vi "LabVIEW.Service.Log Rotating.vi"(6 "description":string, 7 "Command":T1(ring), 8 "error in (no error)":errorcluster caption="Fehler (Eingang, kein Fehler)", 9 "command":string, 10 "status":string, 11 "Pfad":path) -> (0 "error out":errorcluster caption="Fehler (Ausgang)")   [LabVIEW 2026]
uses:
  <vilib>/Utility/config.llb/Write Key (String).vi
  <vilib>/Utility/config.llb/NI_LVConfig.lvlib
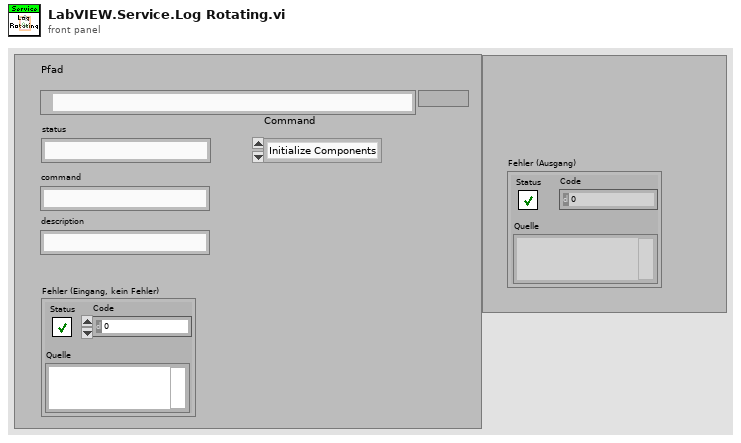
[diagram p1: front panel]
types:
  T1 = enum16{"Initialize Components", "Loging", "Delete Loging"}
  T2 = typedef "NI_LVConfig.lvlib/Config Data RefNum.ctl" = refnum<k1>
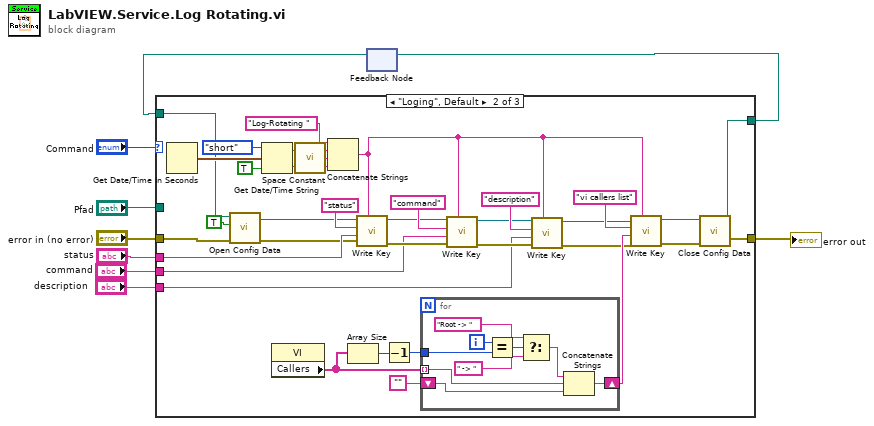
[diagram p0: block diagram]
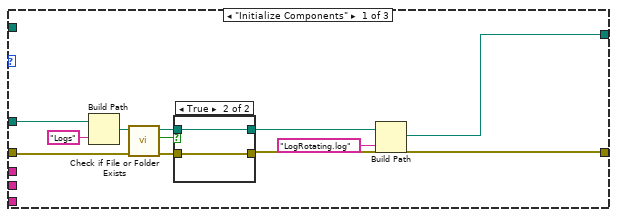
[diagram p2: hidden frame]
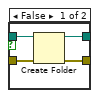
[diagram p3: hidden frame]
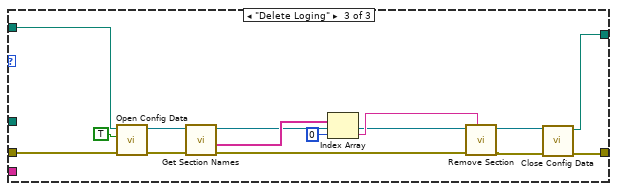
[diagram p4: hidden frame]
diagram:
  n1 = feedback #1() -> (w7:path)  [unwired: 1 in]
  n2 = case shown="\"Loging\", Default" "Command" {
    tunnel: "status" -> [_ w49 _]
    tunnel: [w11 w45 w82] -> w4
    tunnel: w7 -> [_ w42 w81]
    tunnel: "Pfad" -> [w13 _ _]
    tunnel: "error in (no error)" -> [w12 w47 w83]
    tunnel: [w10 w43 w80] -> w3
    tunnel: "command" -> [_ w31 _]
    tunnel: "description" -> [_ w27 _]
    frame "Initialize Components" {
      n3 = Build Path(base path=w13, name or relative path="Logs") -> (appended path=w19:path)
      n4 = call <vilib>:"Check if File or Folder Exists.vi"("error in (no error)"=w12, "path"=w19) -> ("error out"=w20:errorcluster, "file or folder exists?"=w16:bool, "dup path"=w17:path)  [unwired: 7 in]
      n5 = case shown="True" w16 {
        tunnel: w17 -> [w24 w26]
        tunnel: [w23 w25] -> w11
        tunnel: [w22 w26] -> w18
        tunnel: w20 -> [w21 w25]
        frame False {
          n6 = Create Folder(path (use dialog)=w24, error in=w21) -> (created path=w22:path, error out=w23:errorcluster)  [unwired: 1 in, 1 out]
        }
        frame True {
        }
      }
      n7 = Build Path(base path=w18, name or relative path="LogRotating.log") -> (appended path=w10:path)
    }
    frame "Loging", Default {
      n8 = Get Date/Time In Seconds() -> (seconds since 1Jan1904=w60:timestamp)
      n9 = call <vilib>:"Open Config Data.vi"("error in (no error)"=w47, "create file if necessary (T)"=TRUE, "configuration file path"=w42) -> ("error out"=w38:errorcluster, "refnum"=w39:T2)  [unwired: 6 in, 1 out]
      n10 = Get Date/Time String(date format (0)=enum16{"short", "long", "abbreviated"}."short", seconds (now)=w60, want seconds? (F)=TRUE ("Angabe von Sekunden? (F)")) -> (date string=w59:string, time string=w57:string)
      n11 = property class="VI"() -> ("Callers"=w52:string[])  [unwired: 2 in, 2 out]
      n12 = call <vilib>:"Space Constant.vi"() -> ("String"=w58:string)
      n13 = Concatenate Strings("Log-Rotating " ("string"), w59, w58, w57) -> (w30:string)
      n14 = Array Size(array=w52) -> (size(s)=w51:i32)
      n15 = call-poly <vilib>:"Write Key.vi"("section"=w30, "error in (no error)"=w38, "value"=w49, "key"="status", "refnum"=w39) -> ("error out"=w36:errorcluster, "refnum out"=w35:T2)  [unwired: 4 in, 1 out]
      n16 = Decrement(x=w51) -> (x-1=w50:i32)
      n17 = for {
        tunnel: w52 -> [w69] mode=indexing
        shift-right: [w70] -> w53
        shift-left: "" -> [w68]
        tunnel: w50 -> [w63]
        i -> [w64]
        n18 = Equal?(x=w64, y=w63) -> (x = y?=w62:bool)
        n19 = Select(t="Root -> " ("string"), s=w62, f=" -> " ("string")) -> (s? t:f=w65:string)
        n20 = Concatenate Strings(w65, w69, w68) -> (w70:string)
      }
      n21 = call-poly <vilib>:"Write Key.vi"("section"=w30, "error in (no error)"=w36, "value"=w31, "key"="command", "refnum"=w35) -> ("error out"=w32:errorcluster, "refnum out"=w33:T2)  [unwired: 4 in, 1 out]
      n22 = call-poly <vilib>:"Write Key.vi"("section"=w30, "error in (no error)"=w32, "value"=w27, "key"="description", "refnum"=w33) -> ("error out"=w28:errorcluster, "refnum out"=w29:T2)  [unwired: 4 in, 1 out]
      n23 = call-poly <vilib>:"Write Key.vi"("section"=w30, "error in (no error)"=w28, "value"=w53, "key"="vi callers list", "refnum"=w29) -> ("error out"=w46:errorcluster, "refnum out"=w44:T2)  [unwired: 4 in, 1 out]
      n24 = call <vilib>:"Close Config Data.vi"("error in (no error)"=w46, "refnum"=w44) -> ("error out"=w45:errorcluster, "file path"=w43:path)  [unwired: 8 in]
    }
    frame "Delete Loging" {
      n25 = call <vilib>:"Open Config Data.vi"("error in (no error)"=w83, "create file if necessary (T)"=TRUE, "configuration file path"=w81) -> ("error out"=w77:errorcluster, "refnum"=w76:T2)  [unwired: 6 in, 1 out]
      n26 = call <vilib>:"Get Section Names.vi"("error in (no error)"=w77, "refnum"=w76) -> ("error out"=w72:errorcluster, "section names"=w75:string[], "refnum out"=w71:T2)  [unwired: 7 in]
      n27 = Index Array(array=w75, index=0 ("Index")) -> (element=w73:string)
      n28 = call <vilib>:"Remove Section.vi"("section"=w73, "error in (no error)"=w72, "refnum"=w71) -> ("error out"=w79:errorcluster, "refnum out"=w78:T2)  [unwired: 6 in, 1 out]
      n29 = call <vilib>:"Close Config Data.vi"("error in (no error)"=w79, "refnum"=w78) -> ("error out"=w82:errorcluster, "file path"=w80:path)  [unwired: 8 in]
    }
  }
  "error out" <- w4
  n30 = feedback-in #1(w3) -> ()
